vi "Set_MultiVar_Value.vi"(8 "error in (no error)":errorcluster, 9 "varValue":dbl format="%#_13g", 10 "varName":string, 11 "muExpr in":refnum<class "mupExpr.lvclass">) -> (0 "error out":errorcluster, 3 "muExpr out":refnum<class "mupExpr.lvclass">)   [LabVIEW 2015, in "mupExpr.lvclass"]
doc: "Set the value of the specified variable.\n\nIf the variable is not found, a warning is generated."
uses:
  mupExpr.lvclass
  mupExpr.lvclass/mupExpr.ctl
  mupLib/mupSetVarValue.vi
  <vilib>/Utility/error.llb/Error Cluster From Error Code.vi
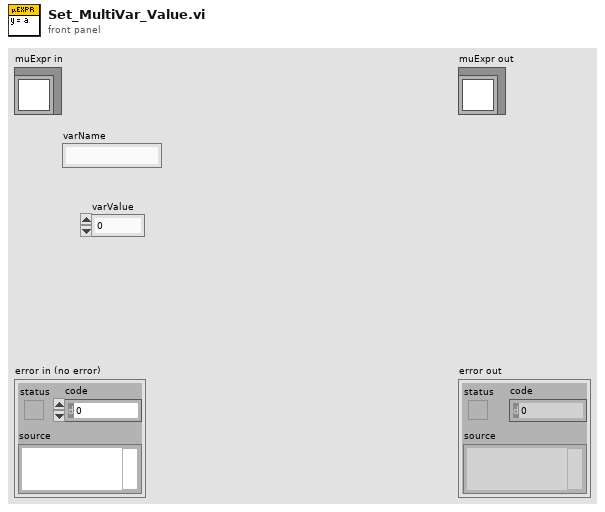
[diagram p1: front panel]
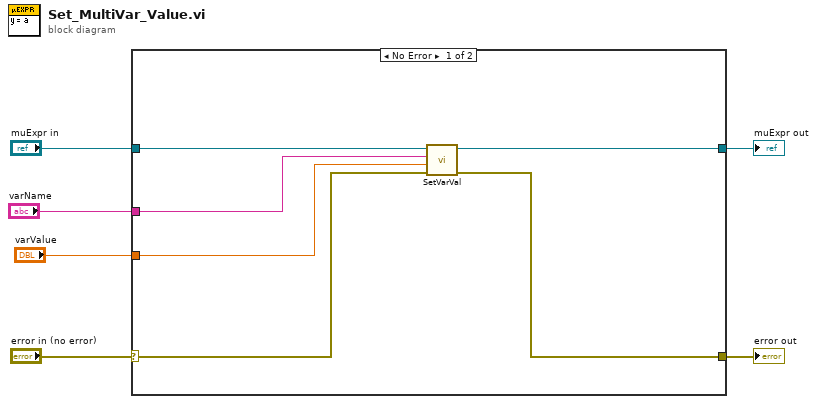
[diagram p0: block diagram]
diagram:
  n1 = case shown="No Error" "error in (no error)" {
    selector: "error in (no error)" -> [w8 w13]
    tunnel: "varValue" -> [w12 _]
    tunnel: "varName" -> [w11 _]
    tunnel: "muExpr in" -> [w10 w14]
    tunnel: [w7 w13] -> w3
    tunnel: [w9 w14] -> w2
    frame No Error {
      n2 = call "SetVarVal.vi"("error in (no error)"=w8, "varValue"=w12, "varName"=w11, "muExpr in"=w10) -> ("error out"=w7:errorcluster, "muExpr out"=w9:refnum<class "mupExpr.lvclass">)  [unwired: 6 in]
    }
    frame Error {
    }
  }
  "error out" <- w3
  "muExpr out" <- w2
